vi "Label.vi"(8 "error in (no error)":errorcluster, 10 "Label":T1, 11 "ITX Commands in":refnum<class "ITX Commands.lvclass">) -> (0 "error out":errorcluster, 3 "ITX Commands out":refnum<class "ITX Commands.lvclass">)   [LabVIEW 2019, in "ITX Commands.lvclass"]
uses:
  ITX Commands.lvclass
  typedefs/Label--cluster.ctl
  ITX Commands.lvclass/ITX Commands.ctl
panel:
  out "resulting string":string
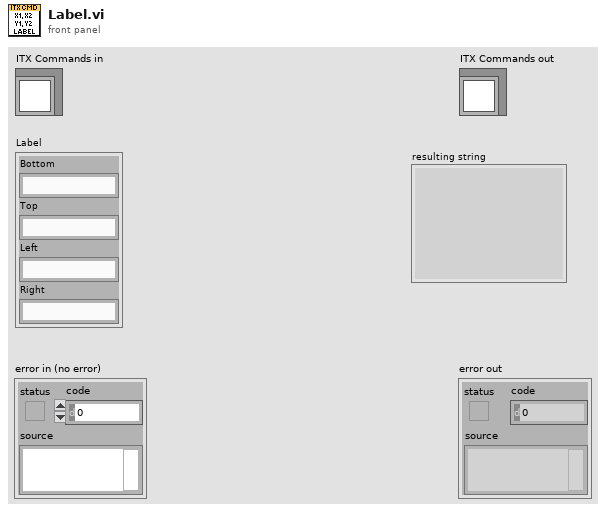
[diagram p1: front panel]
types:
  T1 = typedef "ITX Commands.lvclass/Label--cluster.ctl" = cluster{"Bottom":string, "Top":string, "Left":string, "Right":string}
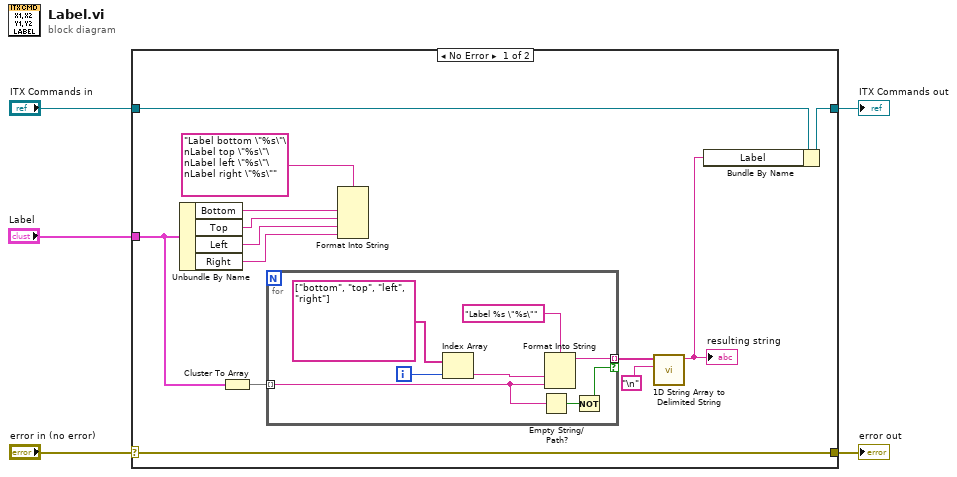
[diagram p0: block diagram]
diagram:
  n1 = case shown="No Error" "error in (no error)" {
    selector: "error in (no error)" -> [w15 w28]
    tunnel: [w15 w28] -> w4
    tunnel: [w16 w27] -> w2
    tunnel: "ITX Commands in" -> [w18 w27]
    tunnel: "Label" -> [w10 _]
    frame No Error {
      n2 = Unbundle By Name(w10) -> ("Bottom"=w11:string, "Top"=w12:string, "Left"=w13:string, "Right"=w14:string)
      n3 = Cluster To Array(cluster=w10) -> (array=w9:string[])
      n4 = for {
        tunnel: w9 -> [w20] mode=indexing
        tunnel: [w24] -> w8 mode=indexing if=w23
        i -> [w19]
        n5 = Index Array(array=string[] ["bottom", "top", "left", "right"], index=w19) -> (element=w22:string)
        n6 = Empty String/Path?(string/path=w20) -> (empty?=w21:bool)
        n7 = Format Into String(format string="Label %s \"%s\"", w22, w20) -> (resulting string=w24:string)  [unwired: 2 in, 1 out]
        n8 = Not(x=w21) -> (.not. x?=w23:bool)
      }
      n9 = Format Into String(format string="Label bottom \"%s\"\nLabel top \"%s\"\nLabel left \"%s\"\nLabel right \"%s\"", w11, w12, w13, w14) -> ()  [unwired: 2 in, 2 out]
      n10 = call <vilib>:"1D String Array to Delimited String.vi"("delimiter"="\n", "string array"=w8) -> ("delimited string"=w6:string)  [unwired: 9 in]
      "resulting string" <- w6
      n11 = Bundle By Name(cluster=w18, "Label"=w6) -> (w16:refnum<class "ITX Commands.lvclass">)
    }
    frame Error {
    }
  }
  "error out" <- w4
  "ITX Commands out" <- w2
